vi "add one letter.vi"() -> ()   [LabVIEW 2025]
panel:
  in  "OK Button":bool
  out "String 2":string
  in  "String":string
  in  "stop":bool
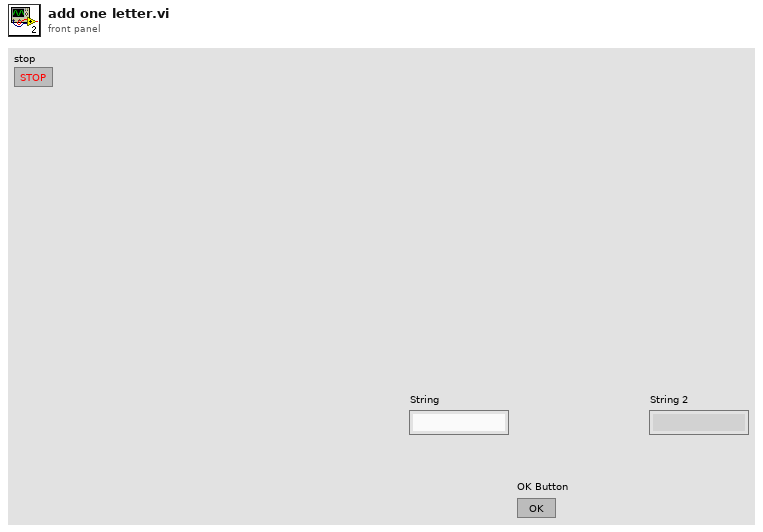
[diagram p1: front panel]
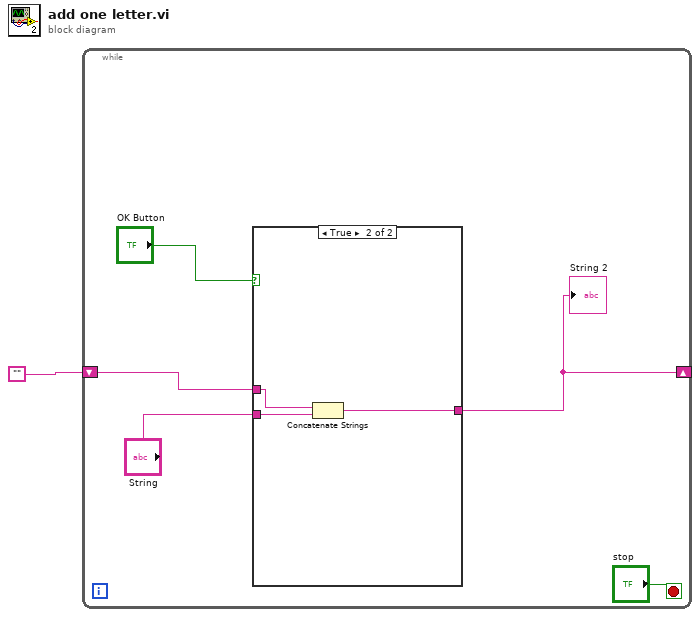
[diagram p0: block diagram]
diagram:
  n1 = while {
    shift-right: [w3] -> _
    shift-left: "" -> [w4]
    stop <- "stop" stop-if-true
    n2 = case shown="True" "OK Button" {
      tunnel: "String" -> [_ w10]
      tunnel: w4 -> [w7 w9]
      tunnel: [w7 w8] -> w3
      frame False {
      }
      frame True {
        n3 = Concatenate Strings(w9, w10) -> (w8:string)
      }
    }
    "String 2" <- w3
  }
